vi "Transmit Dataset.vi"(8 "error in (no error)":errorcluster, 11 "OPC UA in":refnum<class "Abstract.lvclass">=refnum) -> (0 "error out":errorcluster, 3 "OPC UA out":refnum<class "Abstract.lvclass">)   [LabVIEW 2025, in "Abstract.lvclass"]
uses:
  Abstract.lvclass
  Abstract.lvclass/Abstract.ctl
  <vilib>/OPCUA/controls/Write Variant Request.ctl
  <vilib>/OPCUA/controls/NodeId.ctl
  <vilib>/OPCUA/controls/Write Status.ctl
  <vilib>/OPCUA/client/Multiple Write Variant.vi
  <vilib>/OPCUA/NI OPC UA Client.lvlib
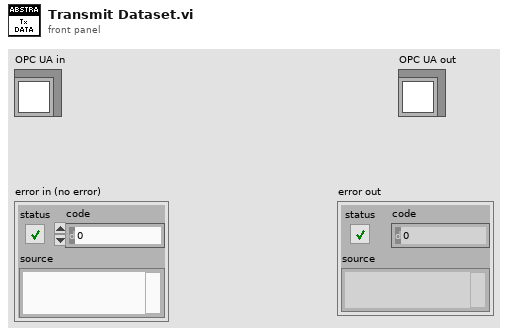
[diagram p1: front panel]
types:
  T1 = typedef "OPC UA Client Refnum.ctl" = refnum<k21>
  T2 = typedef "Write Variant Request.ctl" = cluster{"node ID":T3, "value":variant, "timestamp (current time)":timestamp, "node status":T4}
  T3 = typedef "NodeId.ctl" = string
  T4 = typedef "Write Status.ctl" = u32
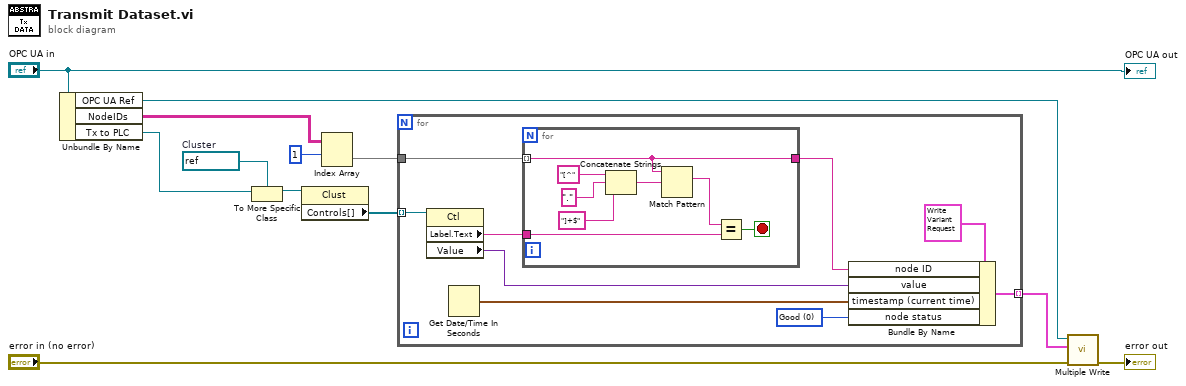
[diagram p0: block diagram]
diagram:
  w8 = refnum<vi> refnum  # Cluster
  n1 = Unbundle By Name("OPC UA in") -> ("OPC UA Ref"=w4:T1, "NodeIDs"=w10:string[][], "Tx to PLC"=w1:refnum<vi>)
  n2 = To More Specific Class(target class=w8, reference=w1) -> (specific class reference=w7:refnum<vi>)  [unwired: 1 in, 1 out]
  n3 = property class="Clust"(reference=w7) -> ("Controls[]"=w6:refnum<vi>[])  [unwired: 1 in, 2 out]
  n4 = Index Array(array=w10, index (row)=1) -> (element=w9:string[])  [unwired: 1 in]
  n5 = for {
    tunnel: w6 -> [w21] mode=indexing
    tunnel: [w17] -> w5 mode=indexing
    tunnel: w9 -> [w19]
    w14 = T4 0 items=["Good"=0, "Uncertain"=1073741824, "Uncertain_InitialValue"=1083310080, "Uncertain_LastUsableValue"=1083179008, "Uncertain_SensorNotAccurate"=1083375616, "Uncertain_EngineeringUnitsExceeded"=1083441152, "Bad"=2147483648, "Bad_NoCommunication"=2150694912, "Bad_NotReadable"=2151284736, "Bad_NotWritable"=2151350272, "Bad_OutOfRange"=2151415808, "Bad_WaitingForInitialData"=2150760448] ("node status")
    n6 = property class="Ctl"(reference=w21) -> ("Label.Text"=w20:string, "Value"=w15:variant)  [unwired: 1 in, 2 out]
    n7 = Get Date/Time In Seconds() -> (seconds since 1Jan1904=w13:timestamp)
    n8 = for {
      tunnel: w20 -> [w29]
      tunnel: w19 -> [w24] mode=indexing
      tunnel: [w24] -> w16
      stop <- w28 stop-if-true
      n9 = Concatenate Strings("[^" ("string"), "." ("Deliminated Char"), "]+$" ("string")) -> (w27:string)
      n10 = Match Pattern(string=w24, regular expression=w27) -> (match substring=w23:string)  [unwired: 1 in, 3 out]
      n11 = Equal?(x=w23, y=w29) -> (x = y?=w28:bool)
    }
    n12 = Bundle By Name(cluster=T2 {"node ID"="", "value"=variant, "timestamp (current time)"=timestamp(0 s since 1904-01-01), "node status"=0} ("request"), "node ID"=w16, "value"=w15, "timestamp (current time)"=w13, "node status"=w14) -> (w17:T2)
  }
  n13 = call-poly <vilib>:"Multiple Write.vi"("error in (no error)"="error in (no error)", "requests"=w5, "OPC UA client refnum in"=w4) -> ("error out"=→"error out":errorcluster)  [unwired: 5 in, 3 out]
  "OPC UA out" <- "OPC UA in"
